vi "Modify Tank.vi"(0 "Original":T1[](array[typedef]), 5 "wheelbase_width":dbl, 11 "error in":errorcluster) -> (4 "original":T1[](array[typedef]), 6 "left":T1[](array[typedef]), 8 "right":T1[](array[typedef]), 15 "error out":errorcluster)   [LabVIEW 2017, in "Pathfinder.lvlib"]
doc: "CAPI void pathfinder_modify_tank(Segment *original, int length, Segment *left, Segment *right, double wheelbase_width);"
uses:
  Pathfinder.lvlib
  Segment.ctl
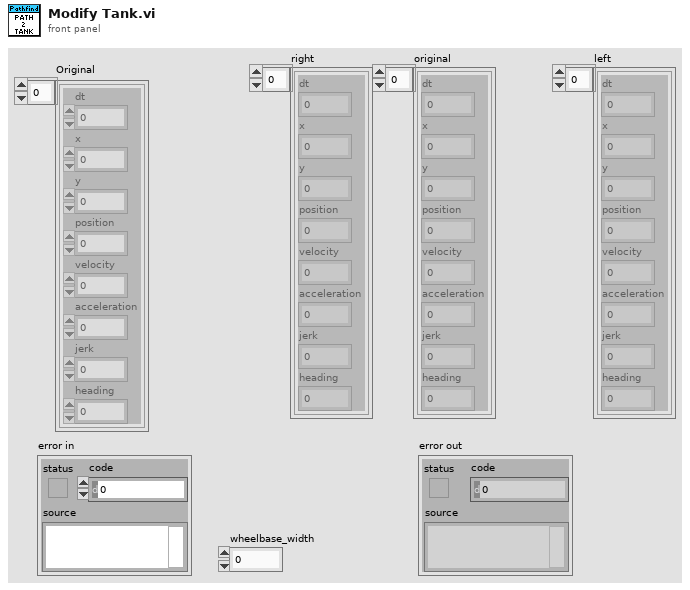
[diagram p1: front panel]
types:
  T1 = typedef "Pathfinder.lvlib/Segment.ctl" = cluster{"dt":dbl, "x":dbl, "y":dbl, "position":dbl, "velocity":dbl, "acceleration":dbl, "jerk":dbl, "heading":dbl}
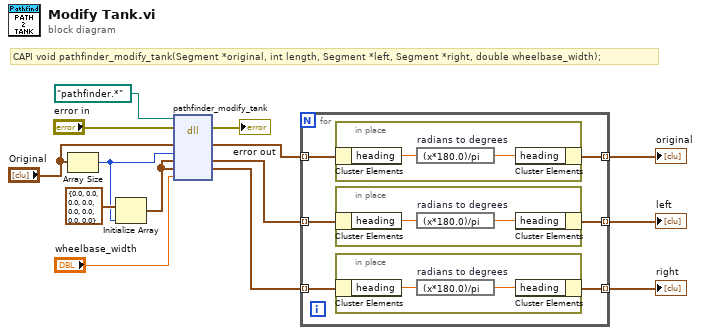
[diagram p0: block diagram]
diagram:
  # "CAPI void pathfinder_modify_tank(Segment *original, int length, Segment *left, Segment *right, double wheelbase_width);"
  n1 = Array Size(array="Original") -> (size(s)=w8:i32)
  n2 = Initialize Array(T1 {"dt"=0.0, "x"=0.0, "y"=0.0, "position"=0.0, "velocity"=0.0, "acceleration"=0.0, "jerk"=0.0, "heading"=0.0} ("segment"), w8) -> (w10:T1[])
  n3 = dll-call lib="?" fn="pathfinder_modify_tank"(path in=path "pathfinder.*", error in="error in", "original"="Original", "length"=w8, "left"=w10, "right"=w10, "wheelbase_width"="wheelbase_width") -> (error out=→"error out":errorcluster, "original"=w6:T1[], "left"=w5:T1[], "right"=w4:T1[])  [unwired: 4 in, 1 out]
  n4 = for {
    tunnel: w6 -> [w20] mode=indexing
    tunnel: w5 -> [w19] mode=indexing
    tunnel: w4 -> [w18] mode=indexing
    tunnel: [w17] -> w3 mode=indexing
    tunnel: [w16] -> w2 mode=indexing
    tunnel: [w15] -> w1 mode=indexing
    n5 = in-place {
      n6 = in-place-cluster #1(w20) -> ("heading"=w26:dbl)
      n7 = expression code="(x*180.0)/pi" "radians to degrees"(w26) -> (w25:dbl)
      n8 = in-place-cluster #1("heading"=w25) -> (w17:T1)
    }
    n9 = in-place {
      n10 = in-place-cluster #2(w19) -> ("heading"=w24:dbl)
      n11 = expression code="(x*180.0)/pi" "radians to degrees"(w24) -> (w23:dbl)
      n12 = in-place-cluster #2("heading"=w23) -> (w16:T1)
    }
    n13 = in-place {
      n14 = in-place-cluster #3(w18) -> ("heading"=w22:dbl)
      n15 = expression code="(x*180.0)/pi" "radians to degrees"(w22) -> (w21:dbl)
      n16 = in-place-cluster #3("heading"=w21) -> (w15:T1)
    }
  }
  "original" <- w3
  "left" <- w2
  "right" <- w1
